vi "Measurement Logic.vi"() -> ()   [LabVIEW 2021, in "Voltage Measurement.lvlib"]
uses:
  Voltage Measurement.lvlib
  Measurement Configuration.ctl
  <instrlib>/niDMM/nidmm.llb/niDMM Resolution in Digits.ctl
  Measurement Results.ctl
  <vilib>/Plug-In SDKs/Measurements/Measure Call Context/Measure Call Context.lvclass
  d5852009-5e3c-4688-848b-1296980261be.vi
  5b802600-c7a4-4cfa-b28d-4d48926cb27b.vi
  <vilib>/Plug-In SDKs/Sessions/niDMM/NI Session Management niDMM.lvlib
  <vilib>/Plug-In SDKs/Sessions/niDCPower/NI Session Management niDCPower.lvlib
  <vilib>/Plug-In SDKs/Clients/Session Management V1/Session Reservation/Session Reservation.lvclass
panel:
  out "measure call context out":refnum<class "Measure Call Context.lvclass">
  in  "measure call context in":refnum<class "Measure Call Context.lvclass">
  out "measurement results":T1={"Measurement "=0.0, "Signal Out of Range"=FALSE, "Measurement from SMU Str"="Empty", "Waveform Graph"=[0.0]} {"Measurement" format="%.6p"}
  in  "measurement configuration":T2={"Vin SMU Channel"="Lorem ipsum dolor sit", "Range"=1.2, "Resolution in Digits"=0.0, "Voltage Config Str"="", "Current Config Str"="", "Vin SMU Pin"="", "Device Name Pin"=""} {"Resolution in Digits" items=["3 1/2"=3.5, "4 1/2"=4.5, "5 1/2"=5.5, "6 1/2"=6.5, "7 1/2"=7.5]}
  out "error out":errorcluster
  in  "error in":errorcluster
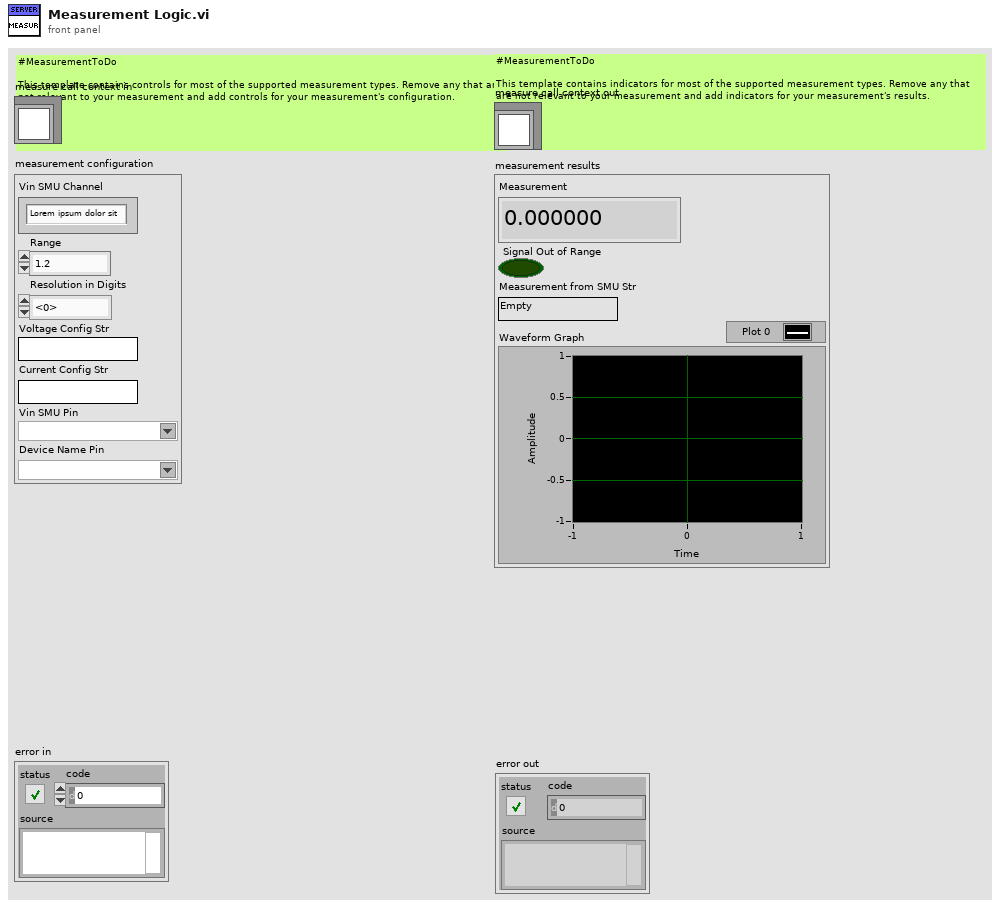
[diagram p1: front panel]
types:
  T1 = typedef "Voltage Measurement.lvlib/Measurement Results.ctl" = cluster{"Measurement ":dbl, "Signal Out of Range":bool, "Measurement from SMU Str":string, "Waveform Graph":dbl[]}
  T2 = typedef "Voltage Measurement.lvlib/Measurement Configuration.ctl" = cluster{"Vin SMU Channel":string, "Range":dbl, "Resolution in Digits":T3, "Voltage Config Str":string, "Current Config Str":string, "Vin SMU Pin":string, "Device Name Pin":string}
  T3 = typedef "niDMM Resolution in Digits.ctl" = dbl
  T4 = typedef "NI Session Management niDMM.lvlib/Connection with Session.ctl" = cluster{"connection":T5, "session":refnum<k15>}
  T5 = typedef "NI Session Management V1 Client.lvlib/Session Reservation.lvclass/Connection.ctl" = cluster{"pin or relay name":string, "site":i32, "instrument type id":string, "channel":string}
  T6 = typedef "NI Session Management niDCPower.lvlib/Connection with Session.ctl" = cluster{"connection":T5, "session":refnum<k15>}
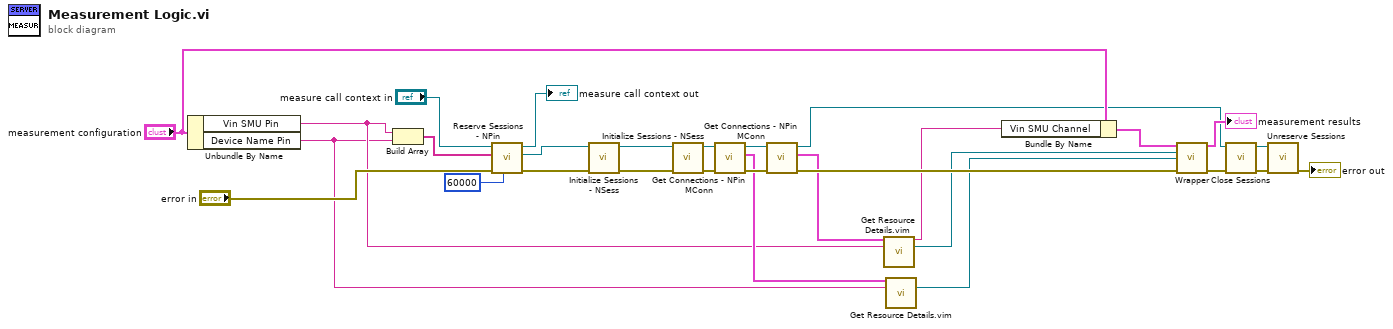
[diagram p0: block diagram]
diagram:
  n1 = Unbundle By Name("measurement configuration") -> ("Vin SMU Pin"=w4:string, "Device Name Pin"=w3:string)
  n2 = Build Array(w4, w3) -> (w25:string[])
  n3 = call <vilib>:"Reserve Sessions - NPin.vi"("timeout (ms)"=60000, "error in"="error in", "pin or relay names"=w25, "measurement context in"="measure call context in") -> ("error out"=w23:errorcluster, "session reservation out"=w22:refnum<class "Session Reservation.lvclass">, "measurement context out"=→"measure call context out":refnum<class "Measure Call Context.lvclass">)  [unwired: 5 in]
  n4 = call <vilib>:"Initialize Sessions - NSess.vi"("error in"=w23, "session reservation in"=w22) -> ("error out"=w21:errorcluster, "session reservation out"=w20:refnum<class "Session Reservation.lvclass">)  [unwired: 6 in, 2 out]
  n5 = call <vilib>:"Initialize Sessions - NSess.vi"("error in"=w21, "session reservation in"=w20) -> ("error out"=w19:errorcluster, "session reservation out"=w18:refnum<class "Session Reservation.lvclass">)  [unwired: 6 in, 2 out]
  n6 = call <vilib>:"Get Connections - NPin MConn.vi"("error in"=w19, "session reservation in"=w18) -> ("error out"=w17:errorcluster, "connections"=w8:T4[], "session reservation out"=w16:refnum<class "Session Reservation.lvclass">)  [unwired: 7 in]
  n7 = call <vilib>:"Get Connections - NPin MConn.vi"("error in"=w17, "session reservation in"=w16) -> ("error out"=w14:errorcluster, "connections"=w6:T6[], "session reservation out"=w12:refnum<class "Session Reservation.lvclass">)  [unwired: 7 in]
  n8 = call "Get Resource Details.vim"("connections"=w6, "Pin Name"=w4) -> ("channel"=w5:string, "session"=w2:refnum<k15>)  [unwired: 12 in]
  n9 = call "Get Resource Details.vim"("connections"=w8, "Pin Name"=w3) -> ("session"=w1:refnum<k15>)  [unwired: 12 in, 1 out]
  n10 = Bundle By Name(cluster="measurement configuration", "Vin SMU Channel"=w5) -> (w7:T2)
  n11 = call "Wrapper.vi"("measurement configuration"=w7, "Vin SMU"=w2, "Device Name"=w1, "error in"=w14) -> ("measurement results"=→"measurement results":T1, "error out"=w13:errorcluster)  [unwired: 10 in]
  n12 = call <vilib>:"Close Sessions.vi"("error in"=w13, "session reservation in"=w12) -> ("error out"=w10:errorcluster, "session reservation out"=w9:refnum<class "Session Reservation.lvclass">)  [unwired: 8 in]
  n13 = call <vilib>:"Unreserve Sessions.vi"("error in"=w10, "session reservation in"=w9) -> ("error out"=→"error out":errorcluster)  [unwired: 9 in]
